vi "Own20261012_FormulaAddOutput.vi"() -> ()   [LabVIEW 2024]
panel:
  out "error out":errorcluster caption="错误输出"
  out "parameter_id":refnum<vi>
  in  "Name":string
  in  "Position":u32
  in  "formula_id":u32
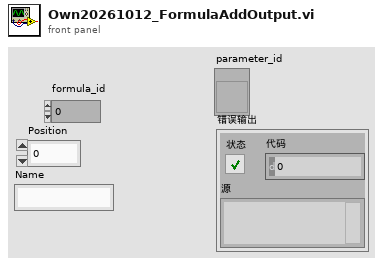
[diagram p1: front panel]
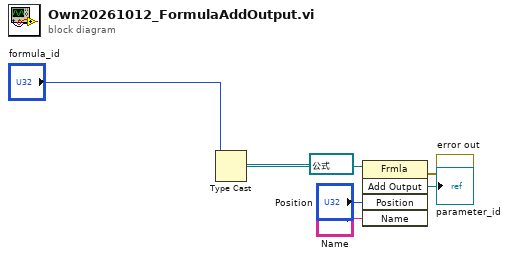
[diagram p0: block diagram]
diagram:
  n1 = Type Cast(type=refnum<vi> refnum ("引用"), x="formula_id") -> (*(type *) &x=w5:refnum<vi>)
  n2 = invoke class="Frmla" method="Add Output"(reference=w5, "Position"="Position", "Name"="Name") -> (error out=→"error out":errorcluster, "Add Output"=→"parameter_id":refnum<vi>)  [unwired: 2 in, 3 out]
